vi "SetHSL.vi"(0 "ColorHLS in":refnum<class "ColorHSL.lvclass">, 5 "H":dbl, 7 "S":dbl, 9 "L":dbl, 11 "error in (no error)":errorcluster) -> (4 "ColorHLS out":refnum<class "ColorHSL.lvclass">, 15 "error out":errorcluster)   [LabVIEW 2021, in "Picture2D.lvlib" / "ColorHSL.lvclass"]
uses:
  ColorHSL.lvclass
  ColorHSL.lvclass/ColorHSL.ctl
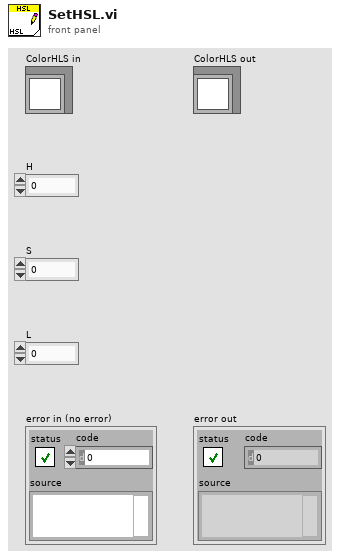
[diagram p1: front panel]
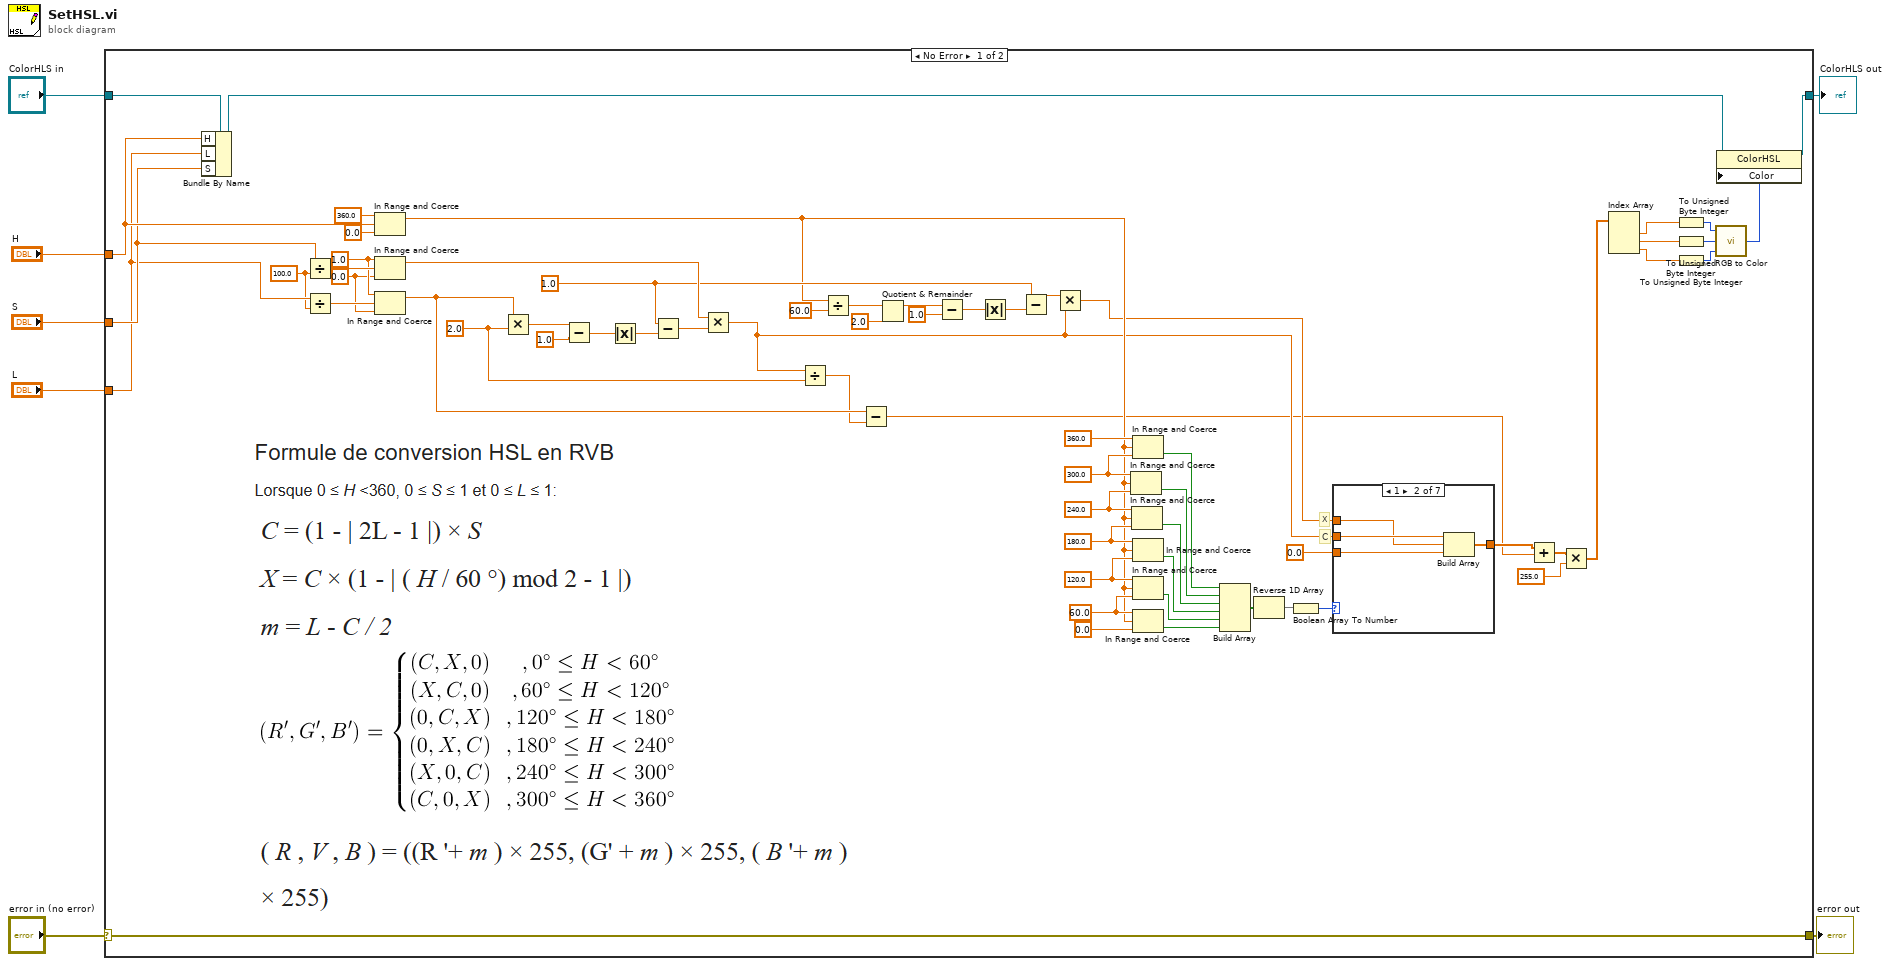
[diagram p0: block diagram]
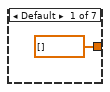
[diagram p2: hidden frame]
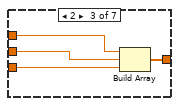
[diagram p3: hidden frame]
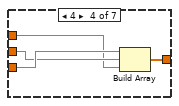
[diagram p4: hidden frame]
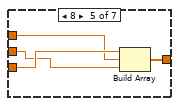
[diagram p5: hidden frame]
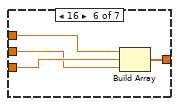
[diagram p6: hidden frame]
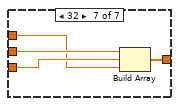
[diagram p7: hidden frame]
diagram:
  n1 = case shown="No Error" "error in (no error)" {
    selector: "error in (no error)" -> [w71 w97]
    tunnel: [w71 w97] -> w6
    tunnel: [w59 w98] -> w4
    tunnel: "ColorHLS in" -> [w70 w98]
    tunnel: "H" -> [w62 _]
    tunnel: "L" -> [w60 _]
    tunnel: "S" -> [w61 _]
    frame No Error {
      w25 = 300.0 ("upper limit")
      w26 = 240.0 ("upper limit")
      w27 = 180.0 ("upper limit")
      w28 = 120.0 ("upper limit")
      w30 = 60.0 ("upper limit")
      w35 = 2.0
      w37 = 1.0
      w51 = 0.0 ("lower limit")
      w52 = 1.0 ("upper limit")
      w57 = 100.0
      # "C"
      # "X"
      n2 = Bundle By Name(cluster=w70, "H"=w62, "L"=w60, "S"=w61) -> (w69:refnum<class "ColorHSL.lvclass">)
      n3 = Divide(x=w61, y=w57) -> (x/y=w54:dbl)
      n4 = Divide(x=w60, y=w57) -> (x/y=w53:dbl)
      n5 = In Range and Coerce(upper limit=360.0, x=w62, lower limit=0.0) -> (coerced(x)=w24:dbl)  [unwired: 1 out]
      n6 = In Range and Coerce(upper limit=w52, x=w54, lower limit=w51) -> (coerced(x)=w46:dbl)  [unwired: 1 out]
      n7 = In Range and Coerce(upper limit=w52, x=w53, lower limit=w51) -> (coerced(x)=w34:dbl)  [unwired: 1 out]
      n8 = Multiply(x=w34, y=w35) -> (x*y=w50:dbl)
      n9 = Subtract(x=w50, y=1.0) -> (x-y=w48:dbl)
      n10 = Absolute Value(x=w48) -> (abs(x)=w47:dbl)
      n11 = Subtract(x=w37, y=w47) -> (x-y=w45:dbl)
      n12 = Multiply(x=w46, y=w45) -> (x*y=w15:dbl)
      n13 = Divide(x=w15, y=w35) -> (x/y=w33:dbl)
      n14 = Divide(x=w24, y=60.0) -> (x/y=w43:dbl)
      n15 = Subtract(x=w34, y=w33) -> (x-y=w11:dbl)
      n16 = Quotient & Remainder(x=w43, y=2.0) -> (x-y*floor(x/y)=w41:dbl)  [unwired: 1 out]
      n17 = Subtract(x=w41, y=1.0) -> (x-y=w39:dbl)
      n18 = Absolute Value(x=w39) -> (abs(x)=w38:dbl)
      n19 = Subtract(x=w37, y=w38) -> (x-y=w36:dbl)
      n20 = Multiply(x=w36, y=w15) -> (x*y=w14:dbl)
      n21 = In Range and Coerce(upper limit=w25, x=w24, lower limit=w26) -> (In Range?=w20:bool)  [unwired: 1 out]
      n22 = In Range and Coerce(upper limit=w26, x=w24, lower limit=w27) -> (In Range?=w21:bool)  [unwired: 1 out]
      n23 = In Range and Coerce(upper limit=360.0, x=w24, lower limit=w25) -> (In Range?=w19:bool)  [unwired: 1 out]
      n24 = In Range and Coerce(upper limit=w27, x=w24, lower limit=w28) -> (In Range?=w22:bool)  [unwired: 1 out]
      n25 = In Range and Coerce(upper limit=w28, x=w24, lower limit=w30) -> (In Range?=w23:bool)  [unwired: 1 out]
      n26 = In Range and Coerce(upper limit=w30, x=w24, lower limit=0.0) -> (In Range?=w32:bool)  [unwired: 1 out]
      n27 = Build Array(w19, w20, w21, w22, w23, w32) -> (w18:bool[])
      n28 = Reverse 1D Array(array=w18) -> (reversed array=w17:bool[])
      n29 = Boolean Array To Number(Boolean array=w17) -> (number=w16:u32)
      n30 = case shown="1" w16 {
        tunnel: w15 -> [_ w76 w80 w82 w85 w89 w94]
        tunnel: w14 -> [_ w75 w77 w81 w86 w91 w93]
        tunnel: 0.0 -> [_ w74 w79 w83 w87 w90 w95]
        tunnel: [dbl[] [] w73 w78 w84 w88 w92 w96] -> w12
        frame Default {
        }
        frame 1 {
          n31 = Build Array(w76, w75, w74) -> (w73:dbl[])
        }
        frame 2 {
          n32 = Build Array(w77, w80, w79) -> (w78:dbl[])
        }
        frame 4 {
          n33 = Build Array(w83, w82, w81) -> (w84:dbl[])
        }
        frame 8 {
          n34 = Build Array(w87, w86, w85) -> (w88:dbl[])
        }
        frame 16 {
          n35 = Build Array(w91, w90, w89) -> (w92:dbl[])
        }
        frame 32 {
          n36 = Build Array(w94, w95, w93) -> (w96:dbl[])
        }
      }
      n37 = Add(x=w12, y=w11) -> (x+y=w10:dbl[])
      n38 = Multiply(x=w10, y=255.0) -> (x*y=w8:dbl[])
      n39 = Index Array(array=w8) -> (element #1=w65:dbl, element #2=w64:dbl, element #3=w63:dbl)  [unwired: 3 in]
      n40 = To Unsigned Byte Integer(number=w65) -> (unsigned 8bit integer=w66:u8)
      n41 = To Unsigned Byte Integer(number=w64) -> (unsigned 8bit integer=w67:u8)
      n42 = To Unsigned Byte Integer(number=w63) -> (unsigned 8bit integer=w68:u8)
      n43 = call <vilib>:"RGB to Color.vi"("B"=w68, "G"=w67, "R"=w66) -> ("Color"=w58:u32)
      n44 = property class="ColorHSL"(reference=w69, "Color"=w58) -> (reference out=w59:refnum<class "ColorHSL.lvclass">)  [unwired: 1 in, 1 out]
    }
    frame Error {
    }
  }
  "error out" <- w6
  "ColorHLS out" <- w4
